vi "Start CLI Interface.vi"(8 "error in (no error)":errorcluster) -> (0 "error out":errorcluster, 1 "Working Directory":path, 2 "Custom Parameters":string[](array[string]), 3 "CLI out":refnum<class "CLI.lvclass">)   [LabVIEW 2015, in "CLI.lvclass"]
doc: "Starts the connection to the command line.\n\n<b>Custom Parameters</b> will return the command line parameters passed for your application."
uses:
  CLI.lvclass
  CLI.lvclass/CLI.ctl
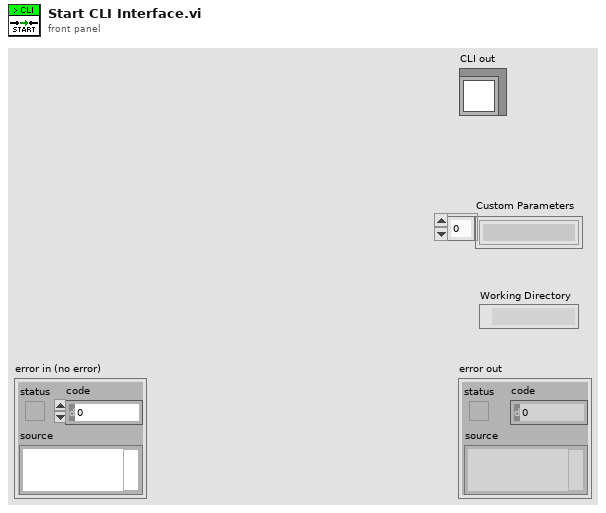
[diagram p1: front panel]
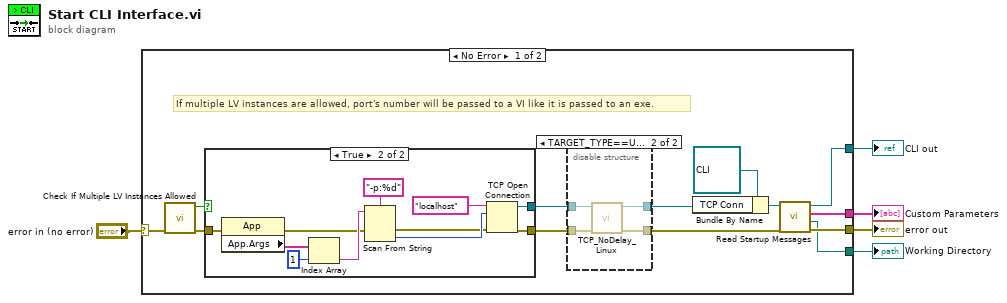
[diagram p0: block diagram]
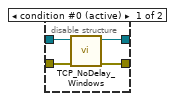
[diagram p2: hidden frame]
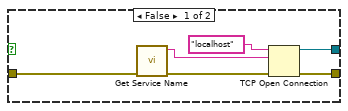
[diagram p3: hidden frame]
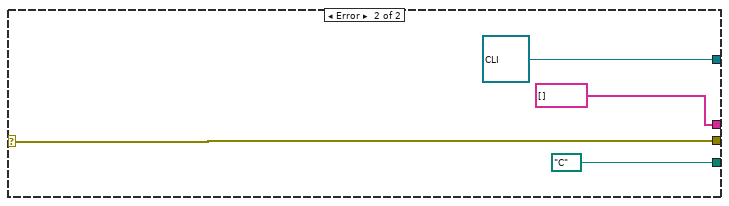
[diagram p4: hidden frame]
diagram:
  n1 = case shown="No Error" "error in (no error)" {
    selector: "error in (no error)" -> [w18 w47]
    tunnel: [w16 w47] -> w4
    tunnel: [w14 refnum<class "CLI.lvclass"> refnum ("CLI in")] -> w3
    tunnel: [w13 string[] []] -> w2
    tunnel: [w12 path "C:/" ("Working Directory")] -> w1
    frame No Error {
      # "If multiple LV instances are allowed, port's number will be passed to a VI like it is passed to an exe."
      n2 = call "Check If Multiple LV Instances Allowed.vi"("error in"=w18) -> ("error out"=w9:errorcluster, "Multiple LV Instances allowed?"=w6:bool)  [unwired: 9 in]
      n3 = case shown="True" w6 {
        tunnel: w9 -> [w29 w35]
        tunnel: [w28 w34] -> w8
        tunnel: [w27 w33] -> w7
        frame False {
          n4 = call "Get Service Name.vi"("error in (no error)"=w29) -> ("error out"=w31:errorcluster, "Service Name"=w32:string)  [unwired: 9 in]
          n5 = TCP Open Connection(address="localhost", remote port or service name=w32, error in (no error)=w31) -> (connection ID=w27:refnum<k5>, error out=w28:errorcluster)  [unwired: 2 in]
        }
        frame True {
          n6 = property class="App"(error in=w35) -> (error out=w36:errorcluster, "App.Args"=w37:string[])  [unwired: 1 in, 1 out]
          n7 = Index Array(array=w37, index=1) -> (element=w41:string)
          n8 = Scan From String(format string="-p:%d", input string=w41, error in=w36) -> (error out=w38:errorcluster, output 1=w40:i32)  [unwired: 2 in, 2 out]
          n9 = TCP Open Connection(address="localhost", remote port or service name=w40, error in (no error)=w38) -> (connection ID=w33:refnum<k5>, error out=w34:errorcluster)  [unwired: 2 in]
        }
      }
      n10 = disable-structure shown="TARGET_TYPE==Unix" {
        disable-tunnel: [w22 w24] -> w11
        disable-tunnel: [w21 w23] -> w10
        disable-tunnel: w8 -> [w20 w25]
        disable-tunnel: w7 -> [w19 w26]
        frame condition #0 (active) {
          n11 = call "TCP_NoDelay_Windows.vi"("error in (no error)"=w20, "connID"=w19) -> ("error out"=w21:errorcluster, "connID 2"=w22:refnum<k5>)  [unwired: 4 in]
        }
        frame condition #1 {
          n12 = call "TCP_NoDelay_Linux.vi"("error in (no error)"=w25, "connID"=w26) -> ("error out"=w23:errorcluster, "connID 2"=w24:refnum<k5>)  [unwired: 4 in]
        }
      }
      n13 = Bundle By Name(cluster=refnum<class "CLI.lvclass"> refnum ("CLI in"), "TCP Conn"=w11) -> (w15:refnum<class "CLI.lvclass">)
      n14 = call "Read Startup Messages.vi"("error in (no error)"=w10, "CLI in"=w15) -> ("error out"=w16:errorcluster, "Working Directory"=w12:path, "Arguments"=w13:string[], "CLI out"=w14:refnum<class "CLI.lvclass">)  [unwired: 6 in]
    }
    frame Error {
    }
  }
  "error out" <- w4
  "CLI out" <- w3
  "Custom Parameters" <- w2
  "Working Directory" <- w1
